vi "LabApp - Analog Input Simulator.vi"(6 "error in":errorcluster, 9 "# channels":i32=8) -> (0 "error out":errorcluster, 2 "Data Out":dbl[](array[numeric]) format="%.2f")   [LabVIEW 2021]
doc: "::: CalcExpress Toolkit :::\nCopyright (c) 2000-2026 Konstantin Shifershteyn. All rights reserved."
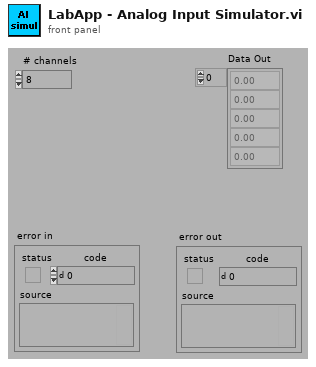
[diagram p1: front panel]
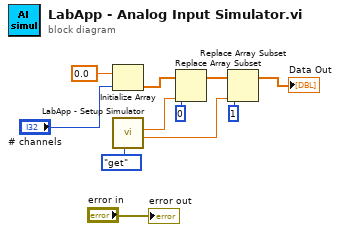
[diagram p0: block diagram]
diagram:
  n1 = Initialize Array(0.0, "# channels") -> (w1:dbl[])
  n2 = call "LabApp - Setup Simulator.vi"("cmd"=enum16{"init", "get", "set"}."get") -> ("param 2"=w2:dbl, "param 1"=w3:dbl)  [unwired: 7 in]
  n3 = Replace Array Subset(array=w1, new element=w3, index=0) -> (w7:dbl[])
  n4 = Replace Array Subset(array=w7, new element=w2, index=1) -> (→"Data Out":dbl[])
  "error out" <- "error in"
